vi "RT Driver VI.vi"(7 "Operation":T1, 11 "Device Reference in":T2 format="%.0x") -> (0 "Error Code":i32)   [LabVIEW 2020]
uses:
  <vilib>/NI/NIVS Inline Async API/_VS Inline Async API/VS Inline Async API/VS Inline Async API.lvclass
  <vilib>/NI VeriStand/Custom Device API/Custom Device API.lvlib
  <vilib>/NI VeriStand/Custom Device Tools/Custom Device Utility Library/Custom Device Utility Library.lvlib
  <vilib>/NI VeriStand/Custom Device API/Get Item Property (Variant).vi
  <vilib>/NI VeriStand/Custom Device API/Data Reference.ctl
  <vilib>/NI VeriStand/Custom Device API/Block Data Reference.ctl
  <vilib>/NI VeriStand/Custom Device API/Custom Device Item Ref.ctl
  <vilib>/NI VeriStand/Custom Device API/Hardware Interface Driver VI Operation.ctl
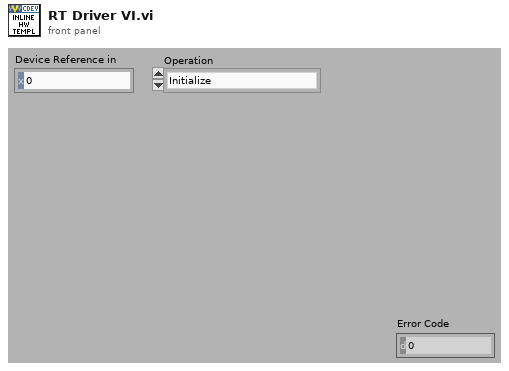
[diagram p1: front panel]
types:
  T1 = typedef "Custom Device API.lvlib/Hardware Interface Driver VI Operation.ctl" = enum16{"Initialize", "Start", "Read Data from HW", "Write Data to HW", "Close"}
  T2 = typedef "Custom Device API.lvlib/Custom Device Item Ref.ctl" = u64
  T3 = cluster{"Async":refnum<class "VS Inline Async API.lvclass">, "Settings":cluster{"Name":string, "Async Init Timeout":u16}}
  T4 = typedef "Custom Device API.lvlib/Block Data Reference.ctl" = cluster{"Data Reference":T5, "Offset":u64, "Length":u64}
  T5 = typedef "Custom Device API.lvlib/Data Reference.ctl" = i32
  T6 = cluster{"Name":string, "Async Init Timeout":u16, "Compiled.InlineAsync.Settings":cluster{"Read":cluster{"Refs":T4[], "Values":dbl[]}[], "Write":cluster{"Refs":T4[], "Values":dbl[]}[], "ReadWrite":cluster{"Refs":T5[], "Values":dbl[], "Reset Values":dbl[]}[], "LUT":variant}}
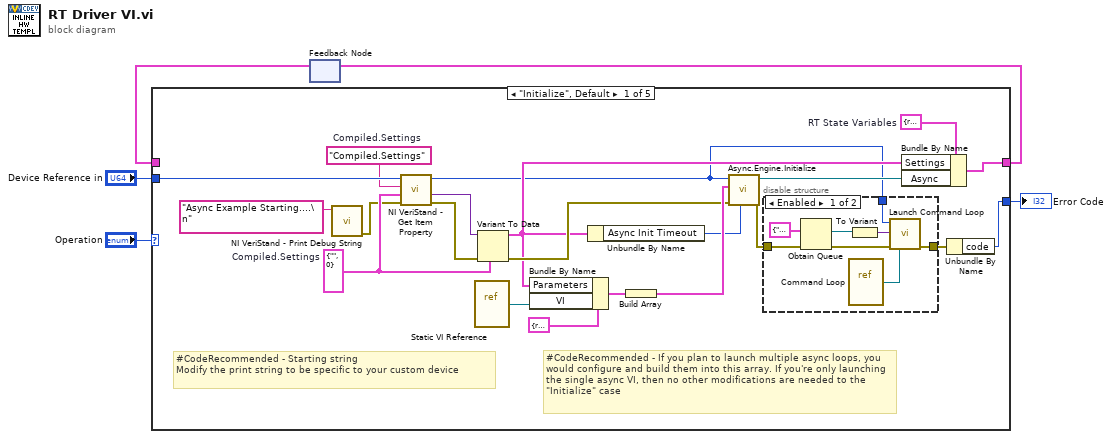
[diagram p0: block diagram]
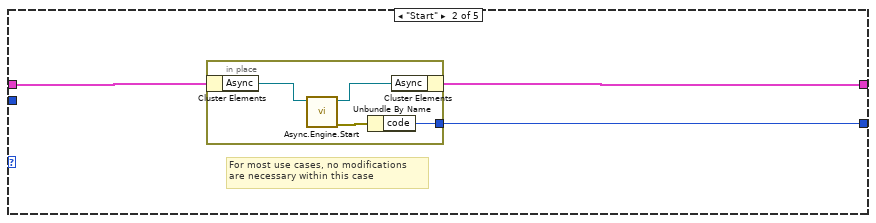
[diagram p3: hidden frame]
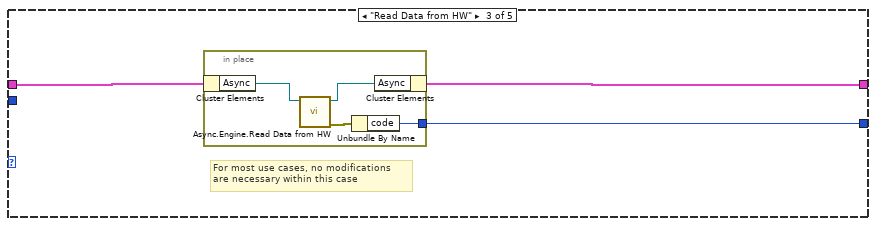
[diagram p4: hidden frame]
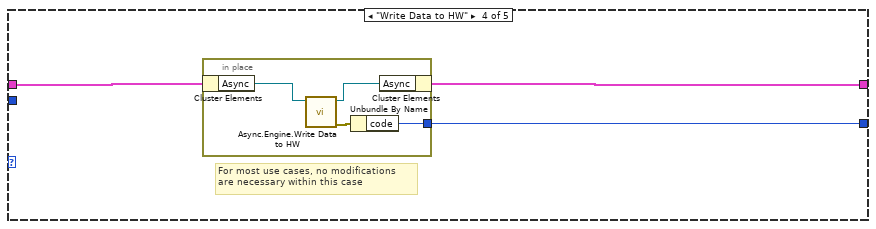
[diagram p5: hidden frame]
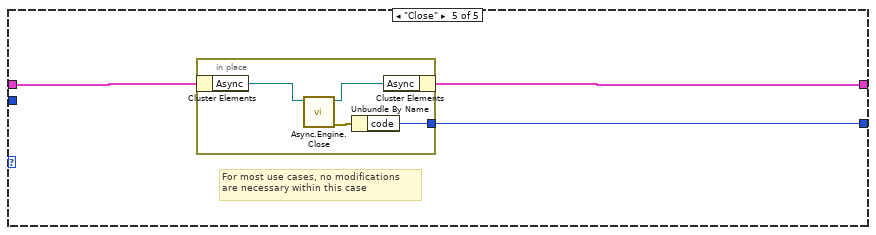
[diagram p6: hidden frame]
diagram:
  n1 = feedback #1() -> (w3:T3)  [unwired: 1 out]
  n2 = case shown="\"Initialize\", Default" "Operation" {
    tunnel: [w24 w37 w43 w50 w58] -> w4
    tunnel: w3 -> [_ w38 w45 w51 w59]
    tunnel: "Device Reference in" -> [w21 _ _ _ _]
    tunnel: [w26 w36 w44 w52 w57] -> w1
    frame "Initialize", Default {
      w16 = T3 {"Async"=refnum, "Settings"={"Name"="", "Async Init Timeout"=0}}  # RT State Variables
      w17 = cluster{"Name":string, "Async Init Timeout":u16} {"Name"="", "Async Init Timeout"=0}  # Compiled.Settings
      w18 = "Compiled.Settings"  # Compiled.Settings
      # "#CodeRecommended - Starting string\nModify the print string to be specific to your custom device"
      # "#CodeRecommended - If you plan to launch multiple async loops, you would configure and build them into this array. If you're only launching the single async VI, then no other modifications are needed to the \"Initialize\" case"
      n3 = call <vilib>:"NI VeriStand - Print Debug String.vi"("Message"="Async Example Starting....\n") -> ("error out"=w13:errorcluster)  [unwired: 10 in]
      n4 = call-poly <vilib>:"NI VeriStand - Get Item Property.vi"("error in (no error)"=w13, "Default Value"=w17, "Property Name"=w18, "Item Ref in"=w21) -> ("error out"=w20:errorcluster, "Value"=w19:variant, "Item Ref out"=w6:T2)  [unwired: 4 in, 1 out]
      n5 = vi-ref "Static VI Reference"() -> ("vi reference"=w11:refnum<vi>)
      n6 = Variant To Data(error in=w20, type=w17, Variant=w19) -> (data=w10:cluster{"Name":string, "Async Init Timeout":u16}, error out=w14:errorcluster)
      n7 = Bundle By Name(cluster=cluster{"VI":refnum<vi>, "Parameters":variant} {"VI"=refnum, "Parameters"=variant} ("Process"), "Parameters"=w10, "VI"=w11) -> (w22:cluster{"VI":refnum<vi>, "Parameters":variant})
      n8 = Unbundle By Name(w10) -> ("Async Init Timeout"=w9:u16)
      n9 = Build Array(w22) -> (w15:cluster{"VI":refnum<vi>, "Parameters":variant}[])
      n10 = call <vilib>:"Async.Engine.Initialize.vi"("Timeout (ms) (5000)"=w9, "error in (no error)"=w14, "Processes"=w15, "Custom Device Ref"=w6) -> ("error out"=w8:errorcluster, "Async"=w25:refnum<class "VS Inline Async API.lvclass">)  [unwired: 6 in]
      n11 = disable-structure shown="Enabled" {
        disable-tunnel: w8 -> [w30 w35]
        disable-tunnel: [w31 w35] -> w7
        disable-tunnel: w6 -> [w27 _]
        frame Enabled {
          n12 = Obtain Queue(element data type=T6 {"Name"="", "Async Init Timeout"=0, "Compiled.InlineAsync.Settings"={"Read"=[], "Write"=[], "ReadWrite"=[], "LUT"=variant}} ("Reconfigure.Settings.ctl"), error in (no error)=w30) -> (queue out=w34:refnum<queue>, error out=w32:errorcluster)  [unwired: 3 in, 1 out]
          n13 = vi-ref "Command Loop.vi"() -> (w29:refnum<vi>)
          n14 = To Variant(anything=w34) -> (Variant=w33:variant)
          n15 = call "Launch Command Loop.vi"("VI Refnum"=w29, "error in"=w32, "Queue Refs"=w33, "Device Reference in"=w27) -> ("error out"=w31:errorcluster)  [unwired: 7 in]
        }
        frame Disabled {
        }
      }
      n16 = Bundle By Name(cluster=w16, "Settings"=w10, "Async"=w25) -> (w24:T3)
      n17 = Unbundle By Name(w7) -> ("code"=w26:i32)
    }
    frame "Start" {
      # "For most use cases, no modifications \nare necessary within this case"
      n18 = in-place {
        in-place-border: [w39] -> w36
        n19 = in-place-cluster #2(w38) -> ("Async"=w42:refnum<class "VS Inline Async API.lvclass">)
        n20 = call <vilib>:"Async.Engine.Start.vi"("VS Inline Async API in"=w42) -> ("error out"=w40:errorcluster, "VS Inline Async API out"=w41:refnum<class "VS Inline Async API.lvclass">)  [unwired: 9 in]
        n21 = Unbundle By Name(w40) -> ("code"=w39:i32)
        n22 = in-place-cluster #2("Async"=w41) -> (w37:T3)
      }
    }
    frame "Read Data from HW" {
      # "For most use cases, no modifications \nare necessary within this case"
      n23 = in-place {
        in-place-border: [w47] -> w44
        n24 = in-place-cluster #3(w45) -> ("Async"=w49:refnum<class "VS Inline Async API.lvclass">)
        n25 = call <vilib>:"Async.Engine.Read Data from HW.vi"("Async in"=w49) -> ("error out"=w46:errorcluster, "Async out"=w48:refnum<class "VS Inline Async API.lvclass">)  [unwired: 9 in]
        n26 = Unbundle By Name(w46) -> ("code"=w47:i32)
        n27 = in-place-cluster #3("Async"=w48) -> (w43:T3)
      }
    }
    frame "Write Data to HW" {
      # "For most use cases, no modifications \nare necessary within this case"
      n28 = in-place {
        in-place-border: [w56] -> w52
        n29 = in-place-cluster #4(w51) -> ("Async"=w54:refnum<class "VS Inline Async API.lvclass">)
        n30 = call <vilib>:"Async.Engine.Write Data to HW.vi"("VS Inline Async API in"=w54) -> ("error out"=w55:errorcluster, "VS Inline Async API out"=w53:refnum<class "VS Inline Async API.lvclass">)  [unwired: 9 in]
        n31 = Unbundle By Name(w55) -> ("code"=w56:i32)
        n32 = in-place-cluster #4("Async"=w53) -> (w50:T3)
      }
    }
    frame "Close" {
      # "For most use cases, no modifications \nare necessary within this case"
      n33 = in-place {
        in-place-border: [w61] -> w57
        n34 = in-place-cluster #5(w59) -> ("Async"=w63:refnum<class "VS Inline Async API.lvclass">)
        n35 = call <vilib>:"Async.Engine.Close.vi"("Async in"=w63) -> ("error out"=w60:errorcluster, "Async out"=w62:refnum<class "VS Inline Async API.lvclass">)  [unwired: 9 in]
        n36 = Unbundle By Name(w60) -> ("code"=w61:i32)
        n37 = in-place-cluster #5("Async"=w62) -> (w58:T3)
      }
    }
  }
  "Error Code" <- w1
  n38 = feedback-in #1(w4) -> ()
